vi "Get possible types.vi"(5 "Class Name":T2) -> (1 "Types":T1[](array[typedef]))   [LabVIEW 2019, in "Language Editor.lvlib"]
doc: "- - -\nCopyright (c) 2026, Merecs Engineering GmbH"
uses:
  Language Editor.lvlib
  type defs/Enum Class Name.ctl
  Language Selection/TypeDefs/Enum Property Type.ctl
  Language Selection/Language Selection.lvlib
panel:
  # "Connector Pane"
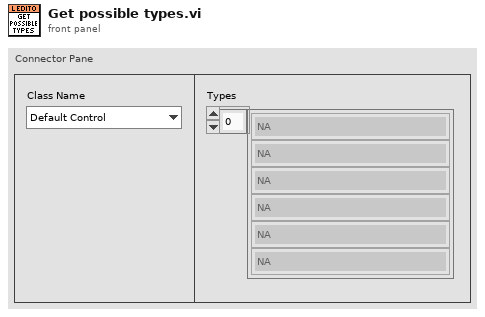
[diagram p1: front panel]
types:
  T1 = typedef "Language Selection.lvlib/Enum Property Type.ctl" = enum16{"NA", "Caption", "String Value", "Boolean Text", "Ring Strings", "1D Array Elements", "2D Array Elements", "(MC)Listbox Header", "(MC)Listbox Items", "Tab Pages Names", "X & Y GraphChart", "Plot Names", "Table Headers", "Table Items", "TipStrip", "Combobox Strings", "Cursor Name", "Tree Col Headers"}
  T2 = typedef "Language Editor.lvlib/Enum Class Name.ctl" = enum16{"Default Control", "Boolean", "ListBox", "Table", "Graph", "Array", "Ring", "String", "TabControl", "ComboBox", "TreeControl"}
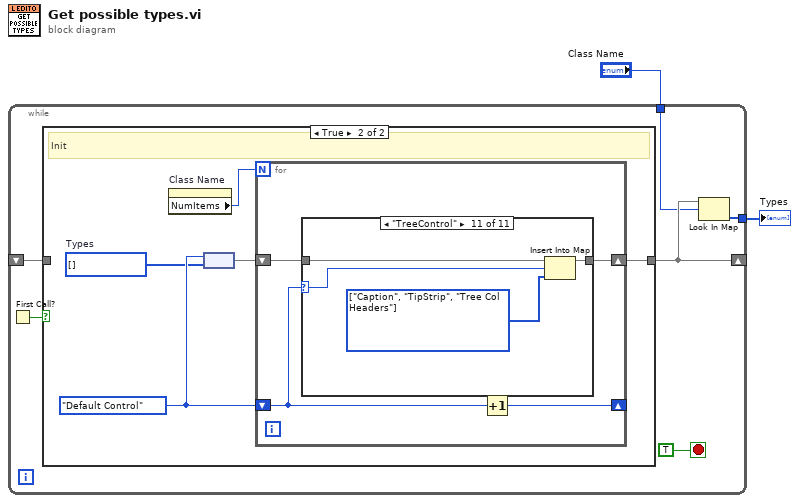
[diagram p0: block diagram]
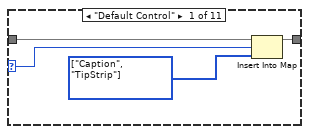
[diagram p3: hidden frame]
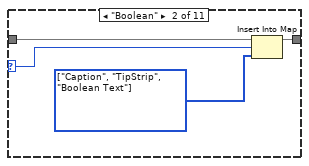
[diagram p4: hidden frame]
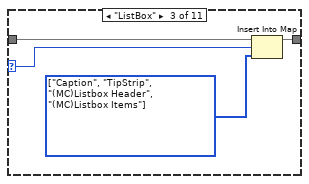
[diagram p5: hidden frame]
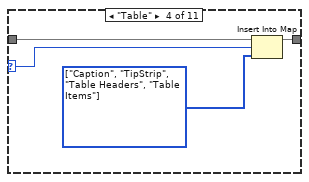
[diagram p6: hidden frame]
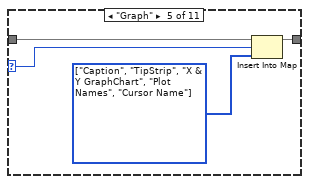
[diagram p7: hidden frame]
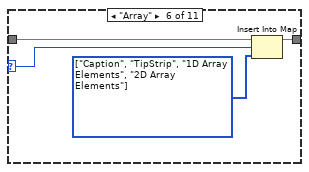
[diagram p8: hidden frame]
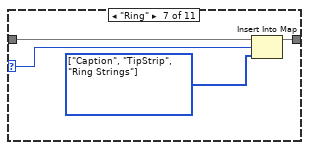
[diagram p9: hidden frame]
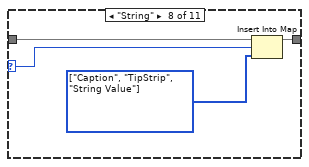
[diagram p10: hidden frame]
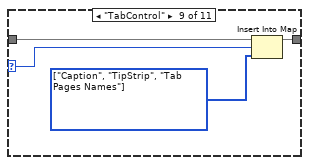
[diagram p11: hidden frame]
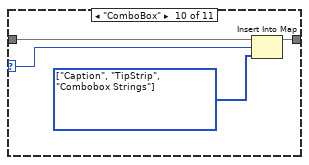
[diagram p12: hidden frame]
diagram:
  n1 = while {
    shift-right: [w8] -> _
    shift-left: _ -> [w4]
    tunnel: "Class Name" -> [w7]
    tunnel: [w6] -> w1
    stop <- TRUE stop-if-true
    n2 = First Call?() -> (First Call?: T/F=w3:bool)
    n3 = case shown="True" w3 {
      tunnel: [w9 w11] -> w8
      tunnel: w4 -> [w9 _]
      frame False {
        # "Get"
      }
      frame True {
        w13 = T1[] [] items=["NA", "Caption", "String Value", "Boolean Text", "Ring Strings", "1D Array Elements", "2D Array Elements", "(MC)Listbox Header", "(MC)Listbox Items", "Tab Pages Names", "X & Y GraphChart", "Plot Names", "Table Headers", "Table Items", "TipStrip", "Combobox Strings", "Cursor Name", "Tree Col Headers"]  # Types
        w14 = Enum_Class_Name."Default Control" ("Class Name")
        # "Init"
        n4 = property on="Class Name" class="Enum (strict)"() -> ("NumItems"=w10:u32)  [unwired: 2 in, 2 out]
        n5 = node(w14, w13) -> (w12:map{T2, T1[]})
        n6 = for {
          N: w10 -> [_]
          shift-right: [w18] -> _
          shift-left: w14 -> [w17]
          shift-right: [w16] -> w11
          shift-left: w12 -> [w15]
          n7 = case shown="\"TreeControl\"" w17 {
            selector: w17 -> [w20 w24 w28 w32 w36 w40 w44 w48 w52 w56 w60]
            tunnel: [w21 w25 w29 w33 w37 w41 w45 w49 w53 w57 w61] -> w16
            tunnel: w15 -> [w22 w26 w30 w34 w38 w42 w46 w50 w54 w58 w62]
            frame "Default Control" {
              w19 = T1[] [enum."Caption", enum."TipStrip"] items=["NA", "Caption", "String Value", "Boolean Text", "Ring Strings", "1D Array Elements", "2D Array Elements", "(MC)Listbox Header", "(MC)Listbox Items", "Tab Pages Names", "X & Y GraphChart", "Plot Names", "Table Headers", "Table Items", "TipStrip", "Combobox Strings", "Cursor Name", "Tree Col Headers"] ("value")
              n8 = Insert Into Map(map in=w22, key=w20, value=w19) -> (map out=w21:map{T2, T1[]})  [unwired: 2 out]
            }
            frame "Boolean" {
              w23 = T1[] [enum."Caption", enum."TipStrip", enum."Boolean Text"] items=["NA", "Caption", "String Value", "Boolean Text", "Ring Strings", "1D Array Elements", "2D Array Elements", "(MC)Listbox Header", "(MC)Listbox Items", "Tab Pages Names", "X & Y GraphChart", "Plot Names", "Table Headers", "Table Items", "TipStrip", "Combobox Strings", "Cursor Name", "Tree Col Headers"] ("value")
              n9 = Insert Into Map(map in=w26, key=w24, value=w23) -> (map out=w25:map{T2, T1[]})  [unwired: 2 out]
            }
            frame "ListBox" {
              w27 = T1[] [enum."Caption", enum."TipStrip", enum."(MC)Listbox Header", enum."(MC)Listbox Items"] items=["NA", "Caption", "String Value", "Boolean Text", "Ring Strings", "1D Array Elements", "2D Array Elements", "(MC)Listbox Header", "(MC)Listbox Items", "Tab Pages Names", "X & Y GraphChart", "Plot Names", "Table Headers", "Table Items", "TipStrip", "Combobox Strings", "Cursor Name", "Tree Col Headers"] ("value")
              n10 = Insert Into Map(map in=w30, key=w28, value=w27) -> (map out=w29:map{T2, T1[]})  [unwired: 2 out]
            }
            frame "Table" {
              w31 = T1[] [enum."Caption", enum."TipStrip", enum."Table Headers", enum."Table Items"] items=["NA", "Caption", "String Value", "Boolean Text", "Ring Strings", "1D Array Elements", "2D Array Elements", "(MC)Listbox Header", "(MC)Listbox Items", "Tab Pages Names", "X & Y GraphChart", "Plot Names", "Table Headers", "Table Items", "TipStrip", "Combobox Strings", "Cursor Name", "Tree Col Headers"] ("value")
              n11 = Insert Into Map(map in=w34, key=w32, value=w31) -> (map out=w33:map{T2, T1[]})  [unwired: 2 out]
            }
            frame "Graph" {
              w35 = T1[] [enum."Caption", enum."TipStrip", enum."X & Y GraphChart", enum."Plot Names", enum."Cursor Name"] items=["NA", "Caption", "String Value", "Boolean Text", "Ring Strings", "1D Array Elements", "2D Array Elements", "(MC)Listbox Header", "(MC)Listbox Items", "Tab Pages Names", "X & Y GraphChart", "Plot Names", "Table Headers", "Table Items", "TipStrip", "Combobox Strings", "Cursor Name", "Tree Col Headers"] ("value")
              n12 = Insert Into Map(map in=w38, key=w36, value=w35) -> (map out=w37:map{T2, T1[]})  [unwired: 2 out]
            }
            frame "Array" {
              w39 = T1[] [enum."Caption", enum."TipStrip", enum."1D Array Elements", enum."2D Array Elements"] items=["NA", "Caption", "String Value", "Boolean Text", "Ring Strings", "1D Array Elements", "2D Array Elements", "(MC)Listbox Header", "(MC)Listbox Items", "Tab Pages Names", "X & Y GraphChart", "Plot Names", "Table Headers", "Table Items", "TipStrip", "Combobox Strings", "Cursor Name", "Tree Col Headers"] ("value")
              n13 = Insert Into Map(map in=w42, key=w40, value=w39) -> (map out=w41:map{T2, T1[]})  [unwired: 2 out]
            }
            frame "Ring" {
              w43 = T1[] [enum."Caption", enum."TipStrip", enum."Ring Strings"] items=["NA", "Caption", "String Value", "Boolean Text", "Ring Strings", "1D Array Elements", "2D Array Elements", "(MC)Listbox Header", "(MC)Listbox Items", "Tab Pages Names", "X & Y GraphChart", "Plot Names", "Table Headers", "Table Items", "TipStrip", "Combobox Strings", "Cursor Name", "Tree Col Headers"] ("value")
              n14 = Insert Into Map(map in=w46, key=w44, value=w43) -> (map out=w45:map{T2, T1[]})  [unwired: 2 out]
            }
            frame "String" {
              w47 = T1[] [enum."Caption", enum."TipStrip", enum."String Value"] items=["NA", "Caption", "String Value", "Boolean Text", "Ring Strings", "1D Array Elements", "2D Array Elements", "(MC)Listbox Header", "(MC)Listbox Items", "Tab Pages Names", "X & Y GraphChart", "Plot Names", "Table Headers", "Table Items", "TipStrip", "Combobox Strings", "Cursor Name", "Tree Col Headers"] ("value")
              n15 = Insert Into Map(map in=w50, key=w48, value=w47) -> (map out=w49:map{T2, T1[]})  [unwired: 2 out]
            }
            frame "TabControl" {
              w51 = T1[] [enum."Caption", enum."TipStrip", enum."Tab Pages Names"] items=["NA", "Caption", "String Value", "Boolean Text", "Ring Strings", "1D Array Elements", "2D Array Elements", "(MC)Listbox Header", "(MC)Listbox Items", "Tab Pages Names", "X & Y GraphChart", "Plot Names", "Table Headers", "Table Items", "TipStrip", "Combobox Strings", "Cursor Name", "Tree Col Headers"] ("value")
              n16 = Insert Into Map(map in=w54, key=w52, value=w51) -> (map out=w53:map{T2, T1[]})  [unwired: 2 out]
            }
            frame "ComboBox" {
              w55 = T1[] [enum."Caption", enum."TipStrip", enum."Combobox Strings"] items=["NA", "Caption", "String Value", "Boolean Text", "Ring Strings", "1D Array Elements", "2D Array Elements", "(MC)Listbox Header", "(MC)Listbox Items", "Tab Pages Names", "X & Y GraphChart", "Plot Names", "Table Headers", "Table Items", "TipStrip", "Combobox Strings", "Cursor Name", "Tree Col Headers"] ("value")
              n17 = Insert Into Map(map in=w58, key=w56, value=w55) -> (map out=w57:map{T2, T1[]})  [unwired: 2 out]
            }
            frame "TreeControl" {
              w59 = T1[] [enum."Caption", enum."TipStrip", enum."Tree Col Headers"] items=["NA", "Caption", "String Value", "Boolean Text", "Ring Strings", "1D Array Elements", "2D Array Elements", "(MC)Listbox Header", "(MC)Listbox Items", "Tab Pages Names", "X & Y GraphChart", "Plot Names", "Table Headers", "Table Items", "TipStrip", "Combobox Strings", "Cursor Name", "Tree Col Headers"] ("value")
              n18 = Insert Into Map(map in=w62, key=w60, value=w59) -> (map out=w61:map{T2, T1[]})  [unwired: 2 out]
            }
          }
          n19 = Increment(x=w17) -> (x+1=w18:T2)
        }
      }
    }
    n20 = Look In Map(map=w8, key=w7) -> (value=w6:T1[])  [unwired: 1 in, 1 out]
  }
  "Types" <- w1
